vi "Indicator-string.vi"(11 "字符串":string) -> (2 "退表名":string, 3 "进表名":string, 5 "为空？":bool)   [LabVIEW 2025]
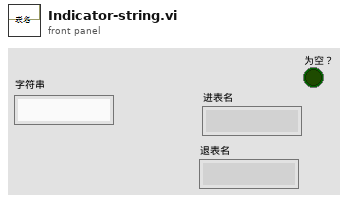
[diagram p1: front panel]
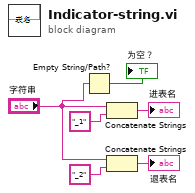
[diagram p0: block diagram]
diagram:
  n1 = Empty String/Path?(string/path="字符串") -> (empty?=→"为空？":bool)
  n2 = Concatenate Strings("字符串", "_1" ("字符串")) -> (→"进表名":string)
  n3 = Concatenate Strings("字符串", "_2" ("字符串")) -> (→"退表名":string)
